vi "Add USB Relay Error Core.vi"(8 "error in (no error)":errorcluster, 10 "String to Append":string, 11 "Error":T1) -> (0 "error out":errorcluster)   [LabVIEW 2021, in "USB Relay Control.lvlib"]
doc: "This reentrant VI contains the error messages. It is called by a wrapper that is inlined for optimal performance. This VI is not inlined to minimize memory impact."
uses:
  USB Relay Control.lvlib
  typedef/Errors.ctl
  <vilib>/CIF Foundation/CIF Utilities/Errors/Errors_CIF_U.lvlib
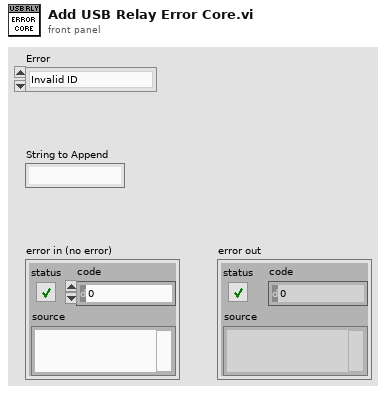
[diagram p1: front panel]
types:
  T1 = typedef "USB Relay Control.lvlib/Errors.ctl" = enum16{"Invalid ID", "Failed to write ID", "Invalid Device"}
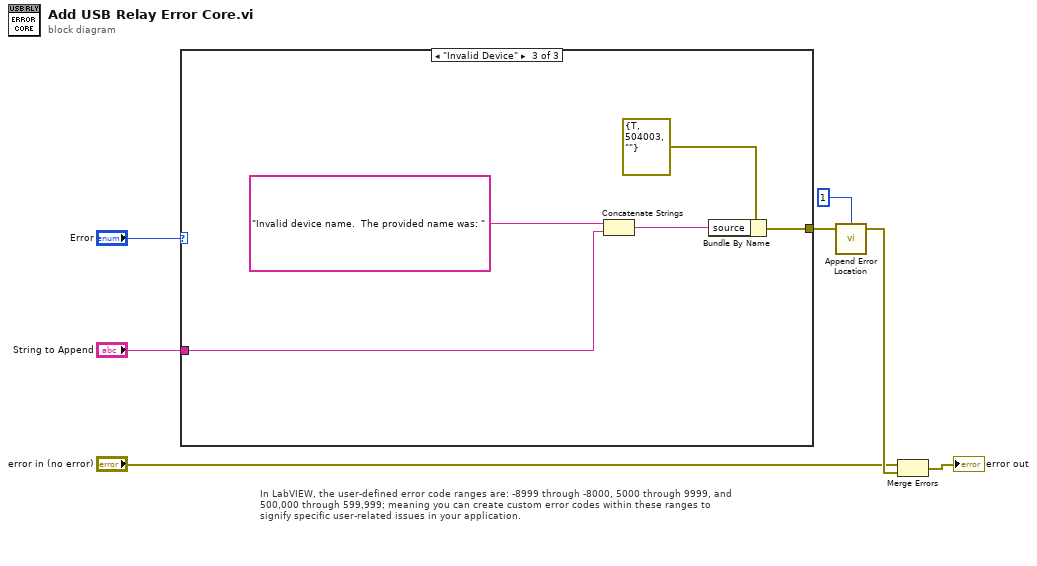
[diagram p0: block diagram]
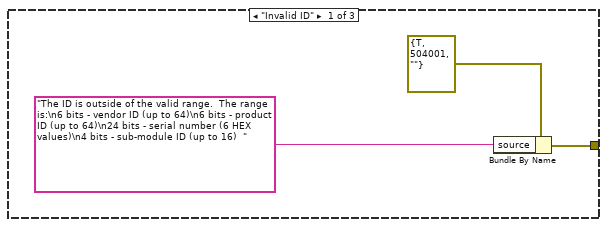
[diagram p2: hidden frame]
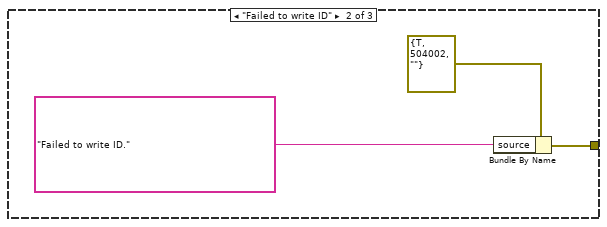
[diagram p3: hidden frame]
diagram:
  # "In LabVIEW, the user-defined error code ranges are: -8999 through -8000, 5000 through 9999, and 500,000 through 599,999; meaning you can create custom error codes within these ranges to signify specific user-related issues in your application."
  n1 = case shown="\"Invalid Device\"" "Error" {
    tunnel: "String to Append" -> [_ _ w15]
    tunnel: [w9 w12 w17] -> w6
    frame "Invalid ID" {
      n2 = Bundle By Name(cluster=errorcluster {"status"=TRUE, "code"=504001, "source"=""} ("Invalid ID"), "source"="The ID is outside of the valid range.  The range is:\n6 bits - vendor ID (up to 64)\n6 bits - product ID (up to 64)\n24 bits - serial number (6 HEX values)\n4 bits - sub-module ID (up to 16)  ") -> (w9:errorcluster)
    }
    frame "Failed to write ID" {
      n3 = Bundle By Name(cluster=errorcluster {"status"=TRUE, "code"=504002, "source"=""} ("Invalid ID"), "source"="Failed to write ID.") -> (w12:errorcluster)
    }
    frame "Invalid Device" {
      n4 = Concatenate Strings("Invalid device name.  The provided name was: " ("source"), w15) -> (w14:string)
      n5 = Bundle By Name(cluster=errorcluster {"status"=TRUE, "code"=504003, "source"=""} ("Invalid ID"), "source"=w14) -> (w17:errorcluster)
    }
  }
  n6 = call <vilib>:"Append Error Location.vi"("error in (no error)"=w6, "Chain Depth"=1) -> ("error out"=w7:errorcluster)  [unwired: 3 in]
  n7 = Merge Errors("error in (no error)", w7) -> (→"error out":errorcluster)
